vi "Read Transport.vi"(8 "error in":errorcluster, 10 "max bytes":u32, 11 "transport session":T2) -> (0 "error out":errorcluster, 1 "bytes read":u32, 2 "data out":string, 3 "transport session out":T2)   [LabVIEW 2015, in "Lengmur_socket.lvlib"]
uses:
  Lengmur_socket.lvlib
  Types/Transport Kind.ctl
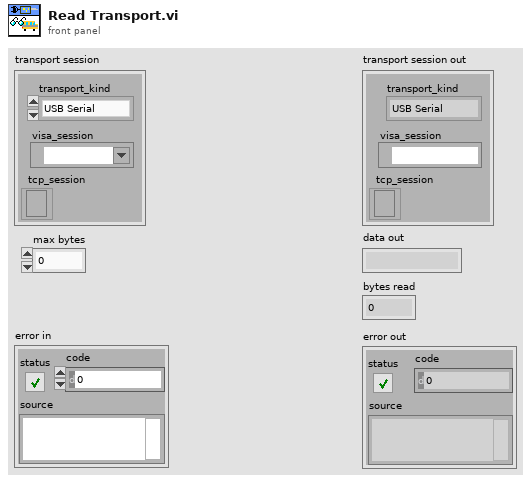
[diagram p1: front panel]
types:
  T1 = typedef "Lengmur_socket.lvlib/Transport Kind.ctl" = enum16{"USB Serial", "Ethernet TCP"}
  T2 = cluster{"transport_kind":T1, "visa_session":refnum<visa-resource-name>, "tcp_session":refnum<k5>}
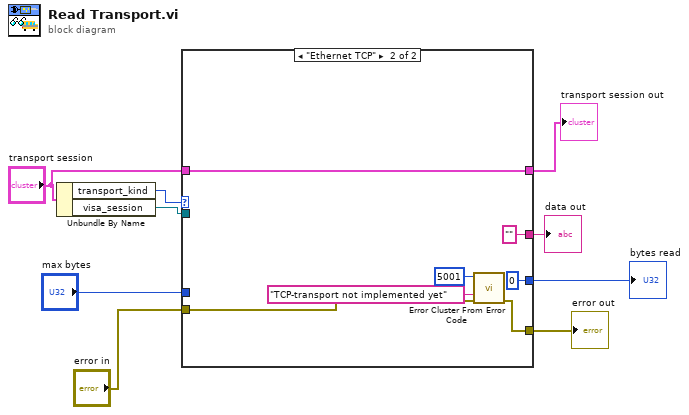
[diagram p0: block diagram]
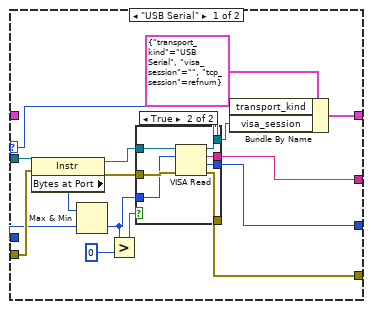
[diagram p2: hidden frame]
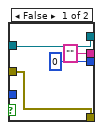
[diagram p3: hidden frame]
diagram:
  n1 = Unbundle By Name("transport session") -> ("transport_kind"=w9:T1, "visa_session"=w6:refnum<visa-resource-name>)
  n2 = case shown="\"Ethernet TCP\"" w9 {
    selector: w9 -> [w21 _]
    tunnel: "error in" -> [w17 w43]
    tunnel: [w25 w40] -> w7
    tunnel: w6 -> [w18 _]
    tunnel: "max bytes" -> [w13 _]
    tunnel: [w24 "" ("read buffer")] -> w4
    tunnel: [w23 u32 0 ("return count")] -> w3
    tunnel: [w19 w37] -> w2
    tunnel: "transport session" -> [_ w37]
    frame "USB Serial" {
      n3 = property class="Instr"(reference=w18, error in=w17) -> (reference out=w16:refnum<visa-resource-name>, error out=w15:errorcluster, "Bytes at Port"=w14:u32)
      n4 = Max & Min(x=w14, y=w13) -> (min(x,y)=w12:u32)  [unwired: 1 out]
      n5 = Greater?(x=w12, y=u32 0) -> (0:w10:bool)
      n6 = case shown="True" w10 {
        tunnel: [w29 w36] -> w25
        tunnel: ["" ("read buffer") w35] -> w24
        tunnel: [u32 0 ("return count") w34] -> w23
        tunnel: [w28 w33] -> w20
        tunnel: w16 -> [w28 w32]
        tunnel: w15 -> [w29 w31]
        tunnel: w12 -> [_ w30]
        frame False {
        }
        frame True {
          n7 = VISA Read(VISA resource name=w32, byte count=w30, error in (no error)=w31) -> (VISA resource name out=w33:refnum<visa-resource-name>, read buffer=w35:string, return count=w34:u32, error out=w36:errorcluster)
        }
      }
      n8 = Bundle By Name(cluster=T2 {"transport_kind"=enum."USB Serial", "visa_session"="", "tcp_session"=refnum} ("transport_session"), "transport_kind"=w21, "visa_session"=w20) -> (w19:T2)
    }
    frame "Ethernet TCP" {
      n9 = call <vilib>:"Error Cluster From Error Code.vi"("error in (no error)"=w43, "error message (\"\")"="TCP-transport not implemented yet" ("error message (\"\")"), "error code (0)"=5001) -> ("error out"=w40:errorcluster)  [unwired: 6 in]
    }
  }
  "transport session out" <- w2
  "data out" <- w4
  "error out" <- w7
  "bytes read" <- w3
